vi "PathPlanner_ConstraintZone_Test.vi"(8 "error in (no error)":errorcluster) -> (0 "error out":errorcluster, 3 "All Passed":bool)   [LabVIEW 2019]
uses:
  <vilib>/Rock Robotics/WPI/ThirdParty/JAS_Junk/TrajLib/Trajectory_Library.lvlib
  <vilib>/Rock Robotics/WPI/ThirdParty/MJansen/PathPlanner/PathPlanner24.lvlib
panel:
  out "Passed 4":bool
  out "Passed 1":bool
  # "JSON Parse"
  # "Getters"
  # "Within Zone"
  # "Overlaps Range"
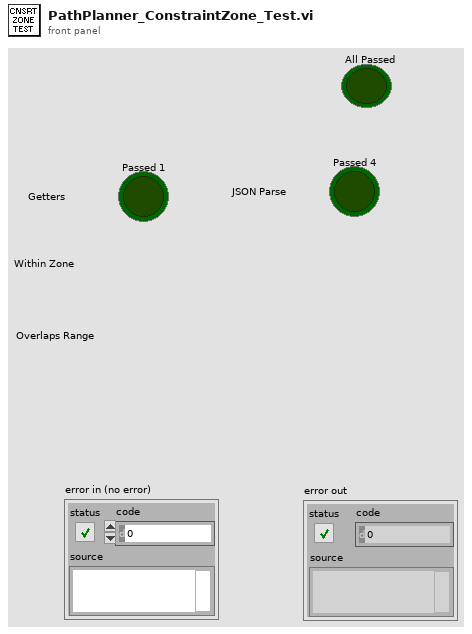
[diagram p1: front panel]
types:
  T1 = typedef "PathPlanner24.lvlib/PathPlannerPathConstraints.ctl" = cluster{"MaxVelocityMps;":dbl, "MaxAccelerationMpsSq;":dbl, "MaxAngularVelRadPsEc;":dbl, "MaxAngularAccRadPSecSq":dbl, "Exists":bool, "Unlimited":bool, "NominalVoltageVolts":dbl}
  T2 = typedef "PathPlanner24.lvlib/PathPlannerConstraintsZone.ctl" = cluster{"minPosition":dbl, "maxPosition":dbl, "Constraints":T1, "Present":bool}
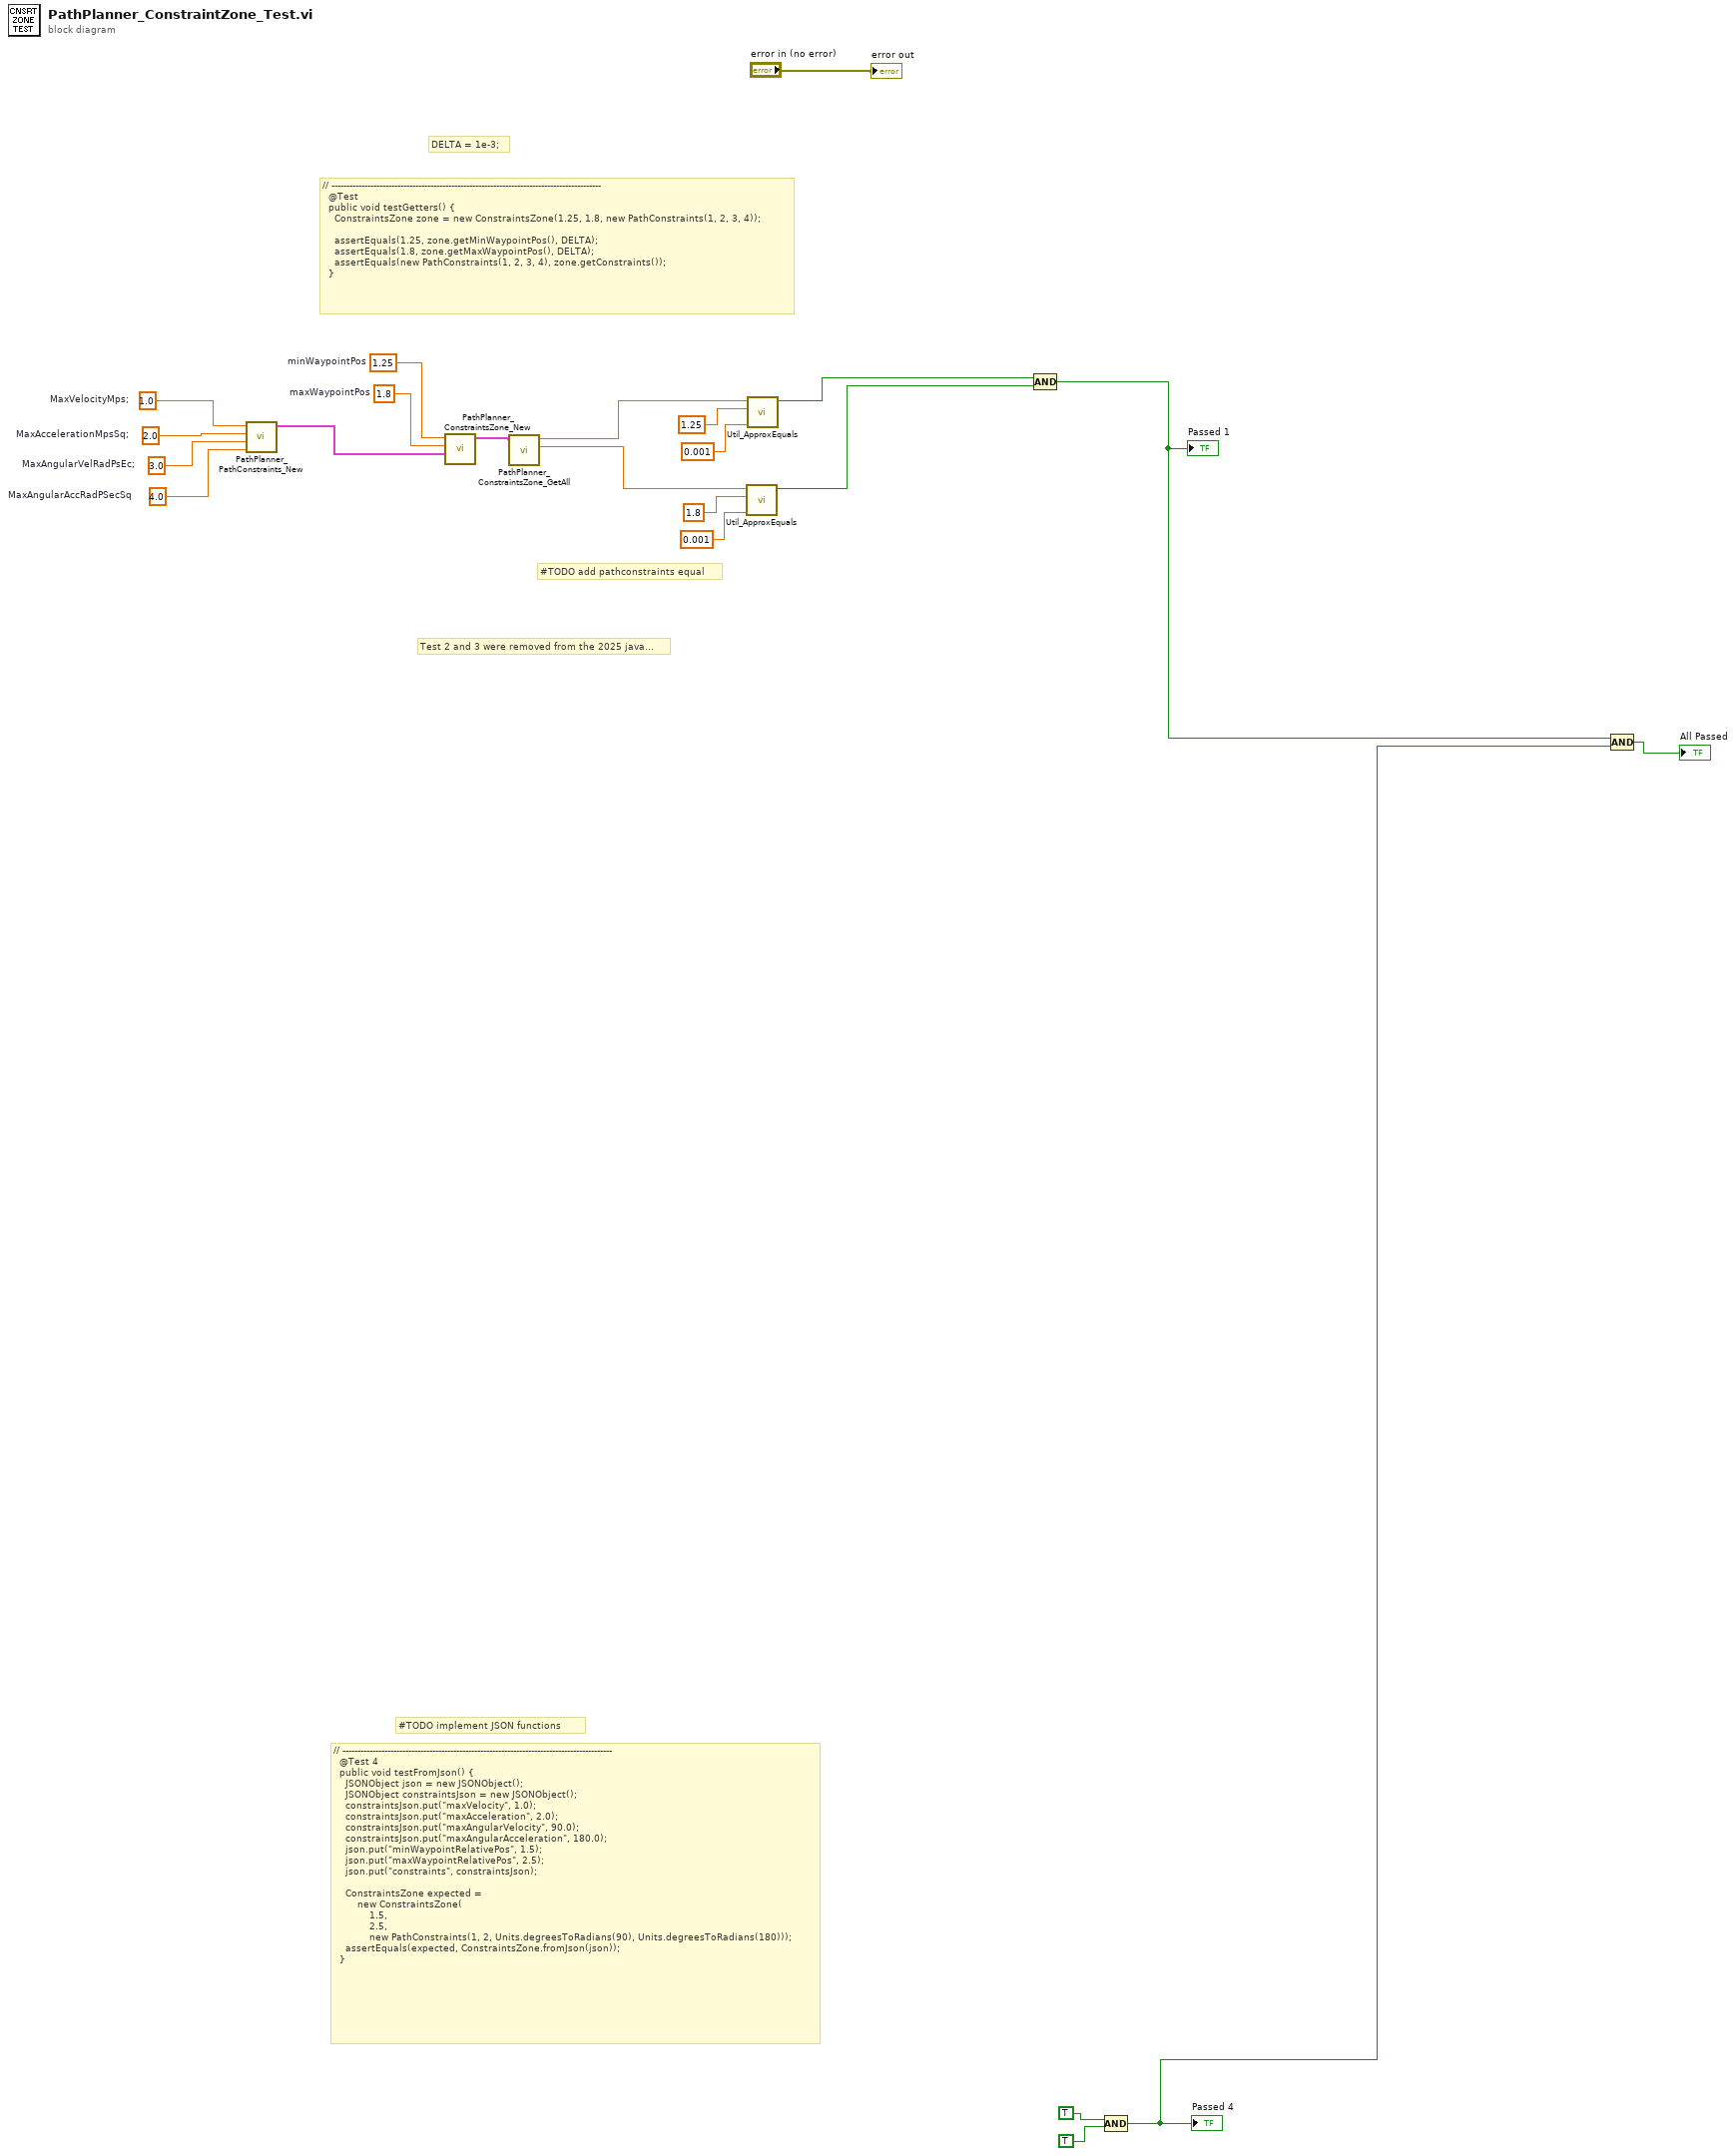
[diagram p0: block diagram]
diagram:
  w13 = 1.8  # maxWaypointPos
  w14 = 1.25  # minWaypointPos
  w15 = 1.0  # MaxVelocityMps;
  w16 = 2.0  # MaxAccelerationMpsSq;
  w17 = 3.0  # MaxAngularVelRadPsEc;
  w18 = 4.0  # MaxAngularAccRadPSecSq
  # "Test 2 and 3 were removed from the 2025 java..."
  # "#TODO implement JSON functions"
  # "// ------------------------------------------------------------------------------------------\n  @Test 4\n  public void testFromJson() {\n    JSONObject json = new JSONObject();\n    JSONObject constraintsJson = new JSONObject();\n    constraintsJson.put(\"maxVelocity\", 1.0);\n    constraintsJson.put(\"maxAcceleration\", 2.0);\n    constraintsJson.put(\"maxAngularVelocity\", 90.0);\n    constraintsJson.put(\"maxAngularAcceleration\", 180.0);\n    json.put(\"minWaypointRelativePos\", 1.5);\n    json.put(\"maxWaypointRelativePos\", 2.5);\n    json.put(\"constraints\", constraintsJson);\n\n    ConstraintsZone expected =\n        new ConstraintsZone(\n            1.5,\n            2.5,\n            new PathConstraints(1, 2, Units.degreesToRadians(90), Units.degreesToRadians(180)));\n    assertEquals(expected, ConstraintsZone.fromJson(json));\n  }"
  # "#TODO add pathconstraints equal"
  # "DELTA = 1e-3;"
  # "// ------------------------------------------------------------------------------------------\n  @Test\n  public void testGetters() {\n    ConstraintsZone zone = new ConstraintsZone(1.25, 1.8, new PathConstraints(1, 2, 3, 4));\n\n    assertEquals(1.25, zone.getMinWaypointPos(), DELTA);\n    assertEquals(1.8, zone.getMaxWaypointPos(), DELTA);\n    assertEquals(new PathConstraints(1, 2, 3, 4), zone.getConstraints());\n  }"
  n1 = call <vilib>:"PathPlanner_PathConstraints_New.vi"("MaxAngularAccRadPSecSq"=w18, "MaxAngularVelRadPsEc;"=w17, "MaxAccelerationMpsSq;"=w16, "MaxVelocityMps;"=w15) -> ("PathPlannerConstraints"=w12:T1)  [unwired: 7 in]
  n2 = call <vilib>:"PathPlanner_ConstraintsZone_New.vi"("Constraints"=w12, "maxPosition"=w13, "minPosition"=w14) -> ("ConstraintsZone"=w11:T2)  [unwired: 8 in]
  n3 = call <vilib>:"PathPlanner_ConstraintsZone_GetAll.vi"("ConstraintsZone"=w11) -> ("maxWaypointPos"=w5:dbl, "minWaypointPos"=w10:dbl)  [unwired: 8 in, 1 out]
  n4 = call <vilib>:"Util_ApproxEquals.vi"("Tolerance"=0.001, "Value 2"=1.8, "Value 1"=w5) -> ("ApproxEquals"=w4:bool)  [unwired: 8 in]
  n5 = call <vilib>:"Util_ApproxEquals.vi"("Tolerance"=0.001, "Value 2"=1.25, "Value 1"=w10) -> ("ApproxEquals"=w20:bool)  [unwired: 8 in]
  n6 = Compound Arithmetic op=AND(w20, w4) -> (w19:bool)
  "Passed 1" <- w19
  n7 = Compound Arithmetic op=AND(TRUE, TRUE) -> (w1:bool)
  "Passed 4" <- w1
  n8 = Compound Arithmetic op=AND(w19, w1) -> (→"All Passed":bool)
  "error out" <- "error in (no error)"
